vi "News Impact.vi"(9 "prices before":dbl[](array[numeric]), 10 "prices now":dbl[](array[numeric]), 11 "stocks":i32[](array[numeric])) -> (3 "affected":T1(array[cluster]))   [LabVIEW 2020, in "Full Featured MCP Server.lvlib"]
doc: "For one news item: every stock it moved, with the move of that stock since just before the news in percent. News that hit every stock return one entry named \"all stocks\" with the average move."
uses:
  Full Featured MCP Server.lvlib
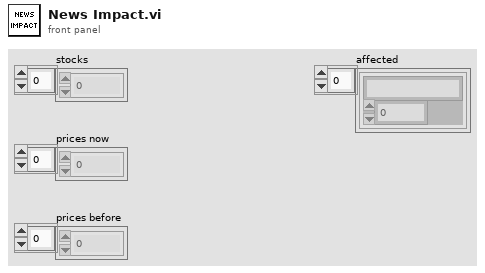
[diagram p1: front panel]
types:
  T1 = cluster{"name":string, "move_since_percent":dbl}[]
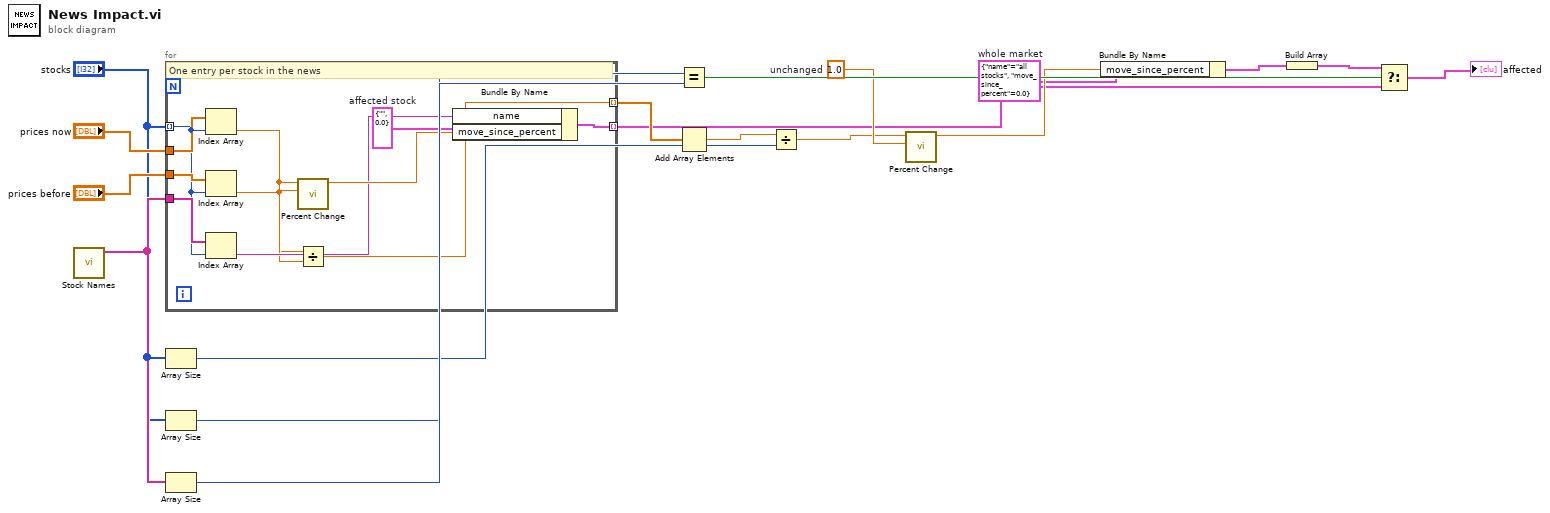
[diagram p0: block diagram]
diagram:
  w11 = 1.0  # unchanged
  w10 = cluster{"name":string, "move_since_percent":dbl} {"name"="all stocks", "move_since_percent"=0.0}  # whole market
  n1 = call "Stock Names.vi"() -> ("names"=w4:string[])  [unwired: 11 in]
  n2 = for {
    tunnel: "stocks" -> [w19] mode=indexing
    tunnel: "prices now" -> [w20]
    tunnel: "prices before" -> [w22]
    tunnel: w4 -> [w25]
    tunnel: [w29] -> w6 mode=indexing
    tunnel: [w28] -> w5 mode=indexing
    w24 = cluster{"name":string, "move_since_percent":dbl} {"name"="", "move_since_percent"=0.0}  # affected stock
    # "One entry per stock in the news"
    n3 = Index Array(array=w20, index=w19) -> (element=w21:dbl)
    n4 = Index Array(array=w22, index=w19) -> (element=w23:dbl)
    n5 = Index Array(array=w25, index=w19) -> (element=w26:string)
    n6 = call "Percent Change.vi"("before"=w23, "now"=w21) -> ("percent"=w27:dbl)  [unwired: 9 in]
    n7 = Divide(x=w21, y=w23) -> (x/y=w29:dbl)
    n8 = Bundle By Name(cluster=w24, "name"=w26, "move_since_percent"=w27) -> (w28:cluster{"name":string, "move_since_percent":dbl})
  }
  n9 = Array Size(array="stocks") -> (size(s)=w8:i32)
  n10 = Array Size(array="stocks") -> (size(s)=w14:i32)
  n11 = Array Size(array=w4) -> (size(s)=w15:i32)
  n12 = Equal?(x=w14, y=w15) -> (x = y?=w16:bool)
  n13 = Add Array Elements(numeric array=w6) -> (sum=w7:dbl)
  n14 = Divide(x=w7, y=w8) -> (x/y=w9:dbl)
  n15 = call "Percent Change.vi"("before"=w11, "now"=w9) -> ("percent"=w12:dbl)  [unwired: 9 in]
  n16 = Bundle By Name(cluster=w10, "move_since_percent"=w12) -> (w13:cluster{"name":string, "move_since_percent":dbl})
  n17 = Build Array(w13) -> (w17:T1)
  n18 = Select(t=w17, s=w16, f=w5) -> (s? t:f=→"affected":T1)
